vi "8-Tap 8-bit Camera with Serial Server(FPGA).vi"() -> ()   [LabVIEW 2013]
doc: "This is the FPGA VI for the 10-Tap 8-Bit Camera with DRAM example. This example demonstrates how to acquire images from a 10-tap, 8-bit, extended configuration, Camera Link camera and transfer the images to the host. This example supports area scan and line scan cameras for both continuous and finite acquisitions.\n\nThis example also demonstrates the use of DRAM as a frame buffer for very high speed acquisitions. Data packing and flow-control are also employed to maximize use of the available DRAM and FIFOs in terms of both memory space and performance.\n\nAdditionally, the example demonstrates the serial server, which allows third-party camera configuration utilities to communicate with the camera using the Camera Link serial interface while this VI is running."
uses:
  Common/CL Signal Mapping.ctl
  Common/CL Configuration.ctl
  FPGA/Sector/Accumulate/Sector Parameter Cluster.ctl
  <vilib>/Platform/TimedLoop/XDataNode/timing_clust.ctl
  <vilib>/Platform/TimedLoop/XDataNode/nitl_modes.ctl
  <vilib>/Platform/TimedLoop/XDataNode/wakeup.ctl
  <vilib>/rvi/eio/common/nirviEmuTemplateMethod_errors.vi
  <vilib>/rvi/Emulation/niFpgaSctlEmulationGetInTimedLoop.vi
  <vilib>/rvi/Emulation/niFpgaEmulationReportErrorSimple.vi
  <vilib>/rvi/Emulation/niFpgaGetClockAttributes.vi
  <vilib>/rvi/Emulation/niFpgaCriticalErrorInLSC.vi
  Common/CL Data to Pixels/8 Tap 8-Bit.vi
  FPGA/Globals/Accumulated Sector Intensity.vi
  <vilib>/rvi/FIFO/Fifo_Resource/nirvififoEmulationWriteFpgaImpl.vi
  <vilib>/rvi/DataTransferAndStorage/Container/Common/niFpgaContainerGetUniqueNameForEmu.vi
  <vilib>/rvi/interface/RandomDataEmulation/nirviRandomDataFPGAFIFO.vi
  <vilib>/rvi/interface/RandomDataEmulation/niFpgaRandomDataHandleErrors.vi
  <vilib>/rvi/FIFO/Fifo_Resource/nirvififoEmulationGetNumberOfElementsToReadFpgaImpl.vi
  <vilib>/rvi/FIFO/Fifo_Resource/nirvififoEmulationGetNumberOfElementsToWriteFpgaImpl.vi
  <vilib>/rvi/FIFO/Fifo_Resource/nirvififoEmulationReadFpgaImpl.vi
  FPGA/Globals/Sector Parameter Global.vi
  <vilib>/rvi/DataTransferAndStorage/Container/Common/niFpgaContainerExecOnDevCompGetState.vi
  <vilib>/rvi/eio/common/nirviEmuReportErrorAndStop.vi
  <vilib>/rvi/Emulation/niFpgaProcessEmulError.vi
  FPGA/Globals/Pixel Location Global.vi
  <vilib>/Platform/TimedLoop/XDataNode/XDataNode.xnode
  <vilib>/eio/EIONode/EIONode.xnode
  <vilib>/rvi/DataTransferAndStorage/Container/XNode/niFpgaContainer.xnode
  <vilib>/rvi/FIFO/Fifo_Resource/nirvififoEmulationWrite.vi
  <vilib>/rvi/interface/RandomDataEmulation/nirviRandomDataFpgaReadWriteTemplate.vi
  <vilib>/rvi/FIFO/Fifo_Resource/nirvififoEmulationGetNumberOfElementsToRead.vi
  <vilib>/rvi/FIFO/Fifo_Resource/nirvififoEmulationGetNumberOfElementsToWrite.vi
  <vilib>/rvi/FIFO/Fifo_Resource/nirvififoEmulationRead.vi
  <vilib>/rvi/FIFO/Fifo_Resource/niFpgaFifoEmulationRefIn.vi
  <vilib>/Platform/TimedLoop/XDataNode/XDNodeRunTimeDep.lvlib
panel:
  out "Host DMA Timeout":bool
  out "Logging?":bool
  in  "Consecutive Sector Threshold":u8
  out "Analysis Ticks":u32
  out "Right Sector Edge":u16
  out "Left Sector Edge":u16
  in  "# of Frames to Average":u8
  in  "Sector Parameters Left":T1={"Start Angle"=0.65740966796875, "End Angle"=0.99468994140625, "Inner Radius"=309, "Outter Radius"=405, "Hinge X"=464, "Hinge Y"=534, "NumWingSectors"=8}
  in  "Sector Parameters Right":T1={"Start Angle"=0.0, "End Angle"=0.4708251953125, "Inner Radius"=309, "Outter Radius"=405, "Hinge X"=685, "Hinge Y"=527, "NumWingSectors"=8}
  in  "Sector Threshold":u8
  in  "[Average BG Intensity]":u8[](array[numeric])=[0, 0, 0, 0, 0, 0, 0, 0, 0, 0, 0, 0, 0, 0, 0, 0, 0, 0, 0, 0, 0, 0, 0, 0, 0, 0, 0, 0, 0, 0, 0, 0]
  in  "X Resolution":u16=1000
  in  "Y Resolution":u16=1000
  in  "Left Start Angle Duty Cycle":fxp<+,8,0>
  in  "Left End Angle Duty Cycle":fxp<+,8,0>
  in  "Right Start Angle Duty Cycle":fxp<+,8,0>
  in  "Right End Angle Duty Cycle":fxp<+,8,0>
  out "Number of Elements to Write Host DMA":u32
  out "Number of Elements to Read Cam Data":u32
  in  "CL Config.Configuration":T2=enum."Full"
  in  "CL Config.Signal Mapping":T3
  in  "CL Config.Line Scan":bool
  in  "CL Config.DVAL Active High":bool=TRUE
  in  "CL Config.LVAL Active High":bool=TRUE
  in  "CL Config.FVAL Active High":bool=TRUE
  in  "CL Config.Spare Active High":bool=TRUE
  in  "Acq Control.Line Scan Height":u32
  in  "Acq Control.Frames To Acq":u32
  in  "Acq Control.Acquire":bool
  in  "Acq Control.Cancel Acq":bool
  in  "Acq Control.Ignore DVAL":bool
  in  "Acq Control.Initialize":bool
  out "Acq Status.Acq In Progress":bool
  out "Acq Status.Clocks Per Line":u32
  out "Acq Status.Frames Acq'd":u32
  out "Acq Status.Lines Per Frame":u32
  out "Acq FIFO Timeout":bool
  out "Acq Status.Initialized":bool
  in  "UART.Baud Rate":u8
  in  "UART.Transmit":bool
  in  "UART.Tx Data":u8[](array[numeric])=[0, 0, 0, 0, 0, 0, 0, 0, 0, 0] format="%02x"
  in  "UART.Set Baud Rate":bool
  in  "UART.Byte Mode":bool=TRUE
  out "UART.Rx Ready":bool
  out "UART.Break Indicator":bool
  out "UART.Framing Error":bool
  out "UART.Overrun Error":bool
  out "UART.Tx Ready":bool
  out "UART.Rx Data":u8 format="%02x"
  in  "UART.Receive":bool
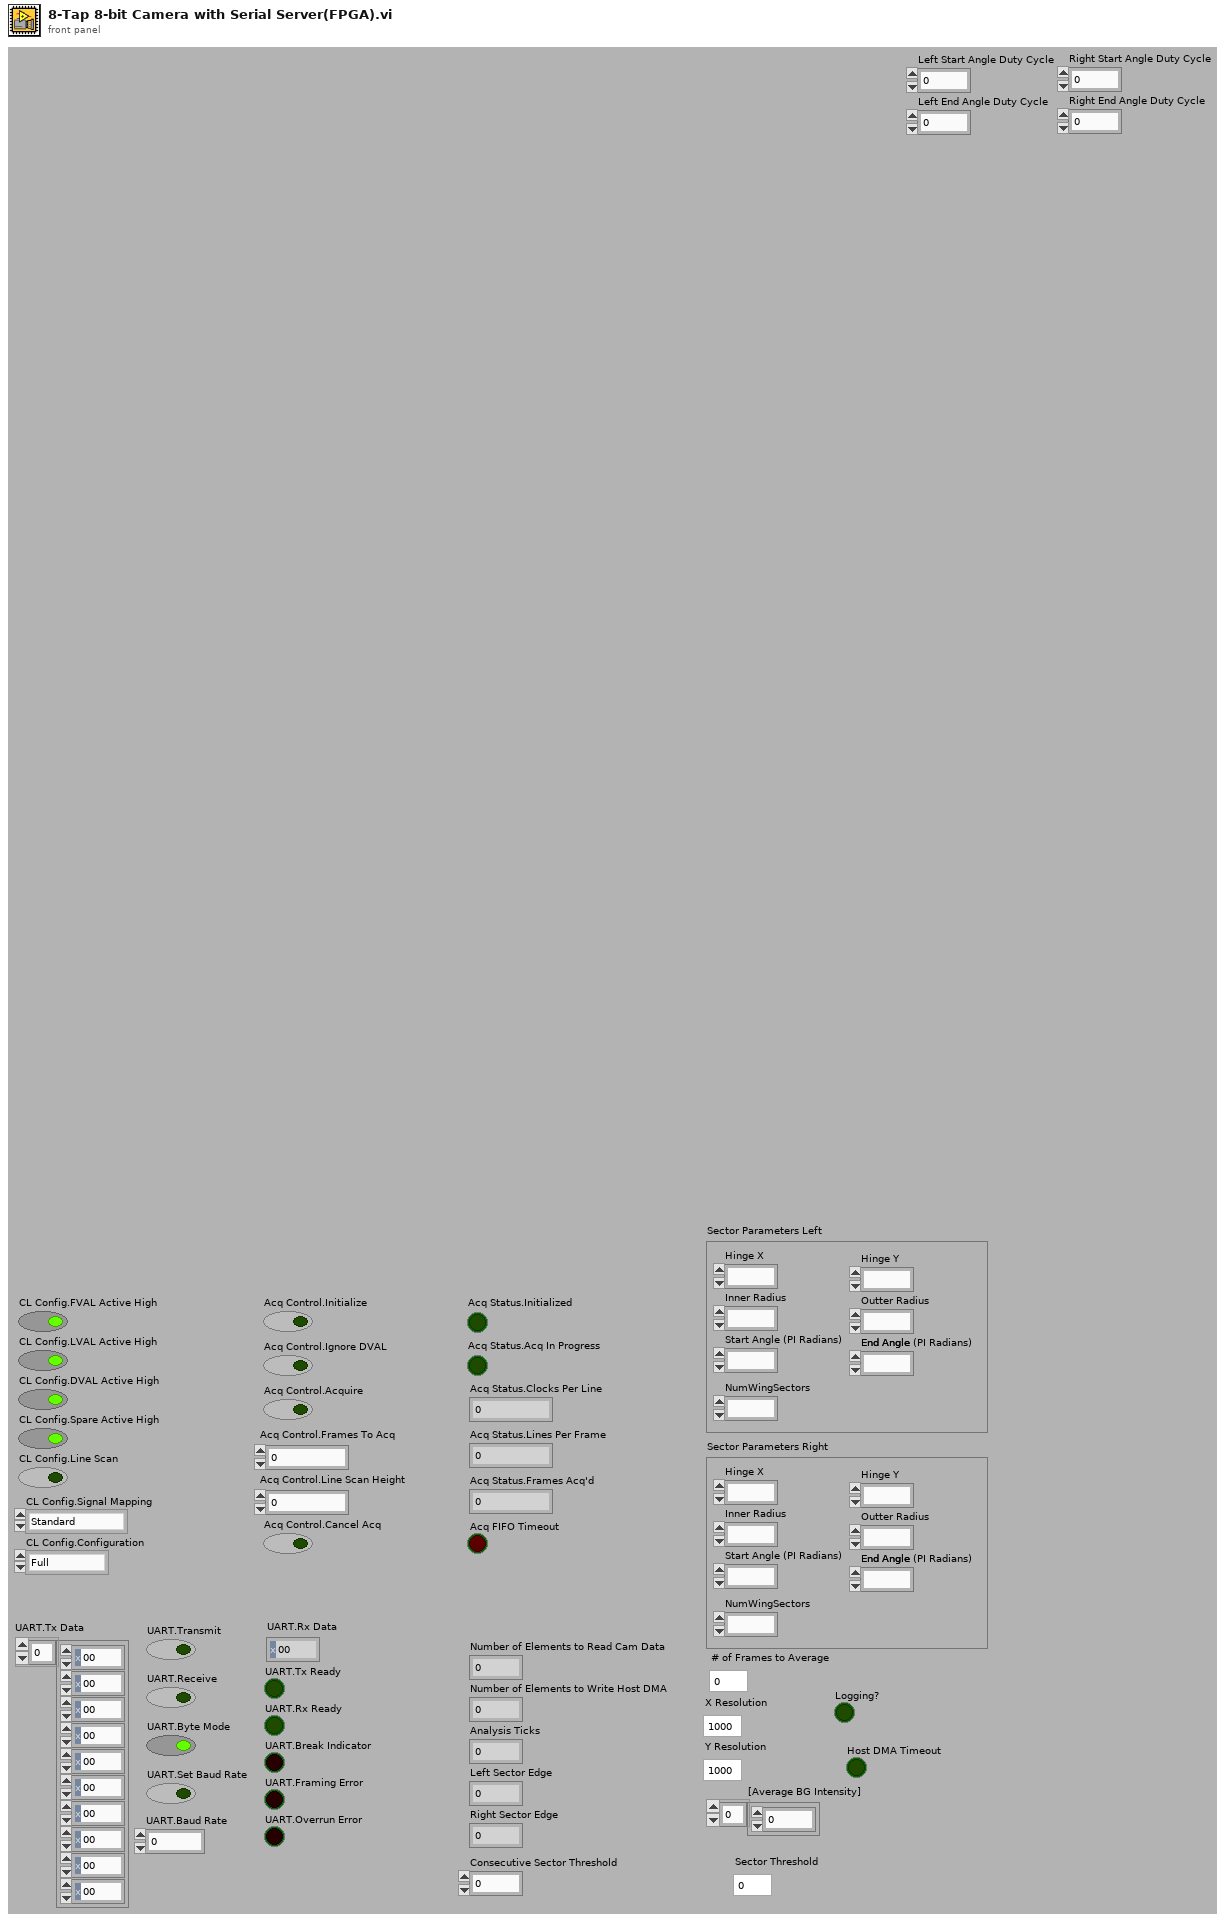
[diagram p1: front panel]
types:
  T1 = typedef "Sector Parameter Cluster.ctl" = cluster{"Start Angle":fxp<+/-,17,2>, "End Angle":fxp<+/-,17,2>, "Inner Radius":u16, "Outter Radius":u16, "Hinge X":u16, "Hinge Y":u16, "NumWingSectors":u8}
  T2 = typedef "CL Configuration.ctl" = enum8{"Base", "Medium", "Full"}
  T3 = typedef "CL Signal Mapping.ctl" = enum8{"Standard", "Basler 10-tap", "Vosskühler 10-tap"}
  T4 = typedef "XDNodeRunTimeDep.lvlib/timing_clust.ctl" = cluster{"Expected End [f-1]":u64, "Actual End [f-1]":u64, "Finished Late? [f-1]":bool, "Expected End [i-1]":u64, "Actual End [i-1]":u64, "Finished Late? [i-1]":bool, "Expected Start [i]":u64, "Actual Start [i]":u64, "Expected Start [f]":u64, "Actual Start [f]":u64, "Source Name":string, "Structure Name":string, "Period":i64, "Deadline":i64, "Offset":i64, "Start":i64, "Priority":i32, "Timeout":i32, "Mode":T5, "Wakeup Reason":T6, "Error":errorcluster, "Source Type":string, "Secondary Source Type":string, "Global End Time":u64, "Global Start Time":u64, "Frame Duration":u64, "Iteration Duration":u64, "Assigned CPU":i32, "I/O Scan Engine Mode":u32}
  T5 = typedef "XDNodeRunTimeDep.lvlib/nitl_modes.ctl" = enum32{"No Change", "Process missed periods, maintain original phase", "Discard missed periods, maintain original phase", "Process missed periods, ignore original phase", "Discard missed periods, ignore original phase"}
  T6 = typedef "XDNodeRunTimeDep.lvlib/wakeup.ctl" = enum32{"Normal", "Aborted", "Asynchronous wakeup", "Timing source error", "Timed loop error", "Timeout"}
  T7 = cluster{"Enables Valid":bool, "Frame Valid":bool, "Line Valid":bool, "Data Valid":bool}
  T8 = cluster{"Pixel 0":u8, "Pixel 1":u8, "Pixel 2":u8, "Pixel 3":u8, "Pixel 4":u8, "Pixel 5":u8, "Pixel 6":u8, "Pixel 7":u8}
  T9 = cluster{"Tx Data":u8[], "Transmit":bool, "Receive":bool, "Byte Mode":bool, "Set Baud Rate":bool, "Baud Rate":u8}
  T10 = cluster{"Rx Data":u8, "Turn Off Transmit":bool, "Turn Off Receive":bool, "Turn Off Set Baud Rate":bool, "Tx Ready":bool, "Rx Ready":bool, "Break Indicator":bool, "Framing Error":bool, "Overrun Error":bool}
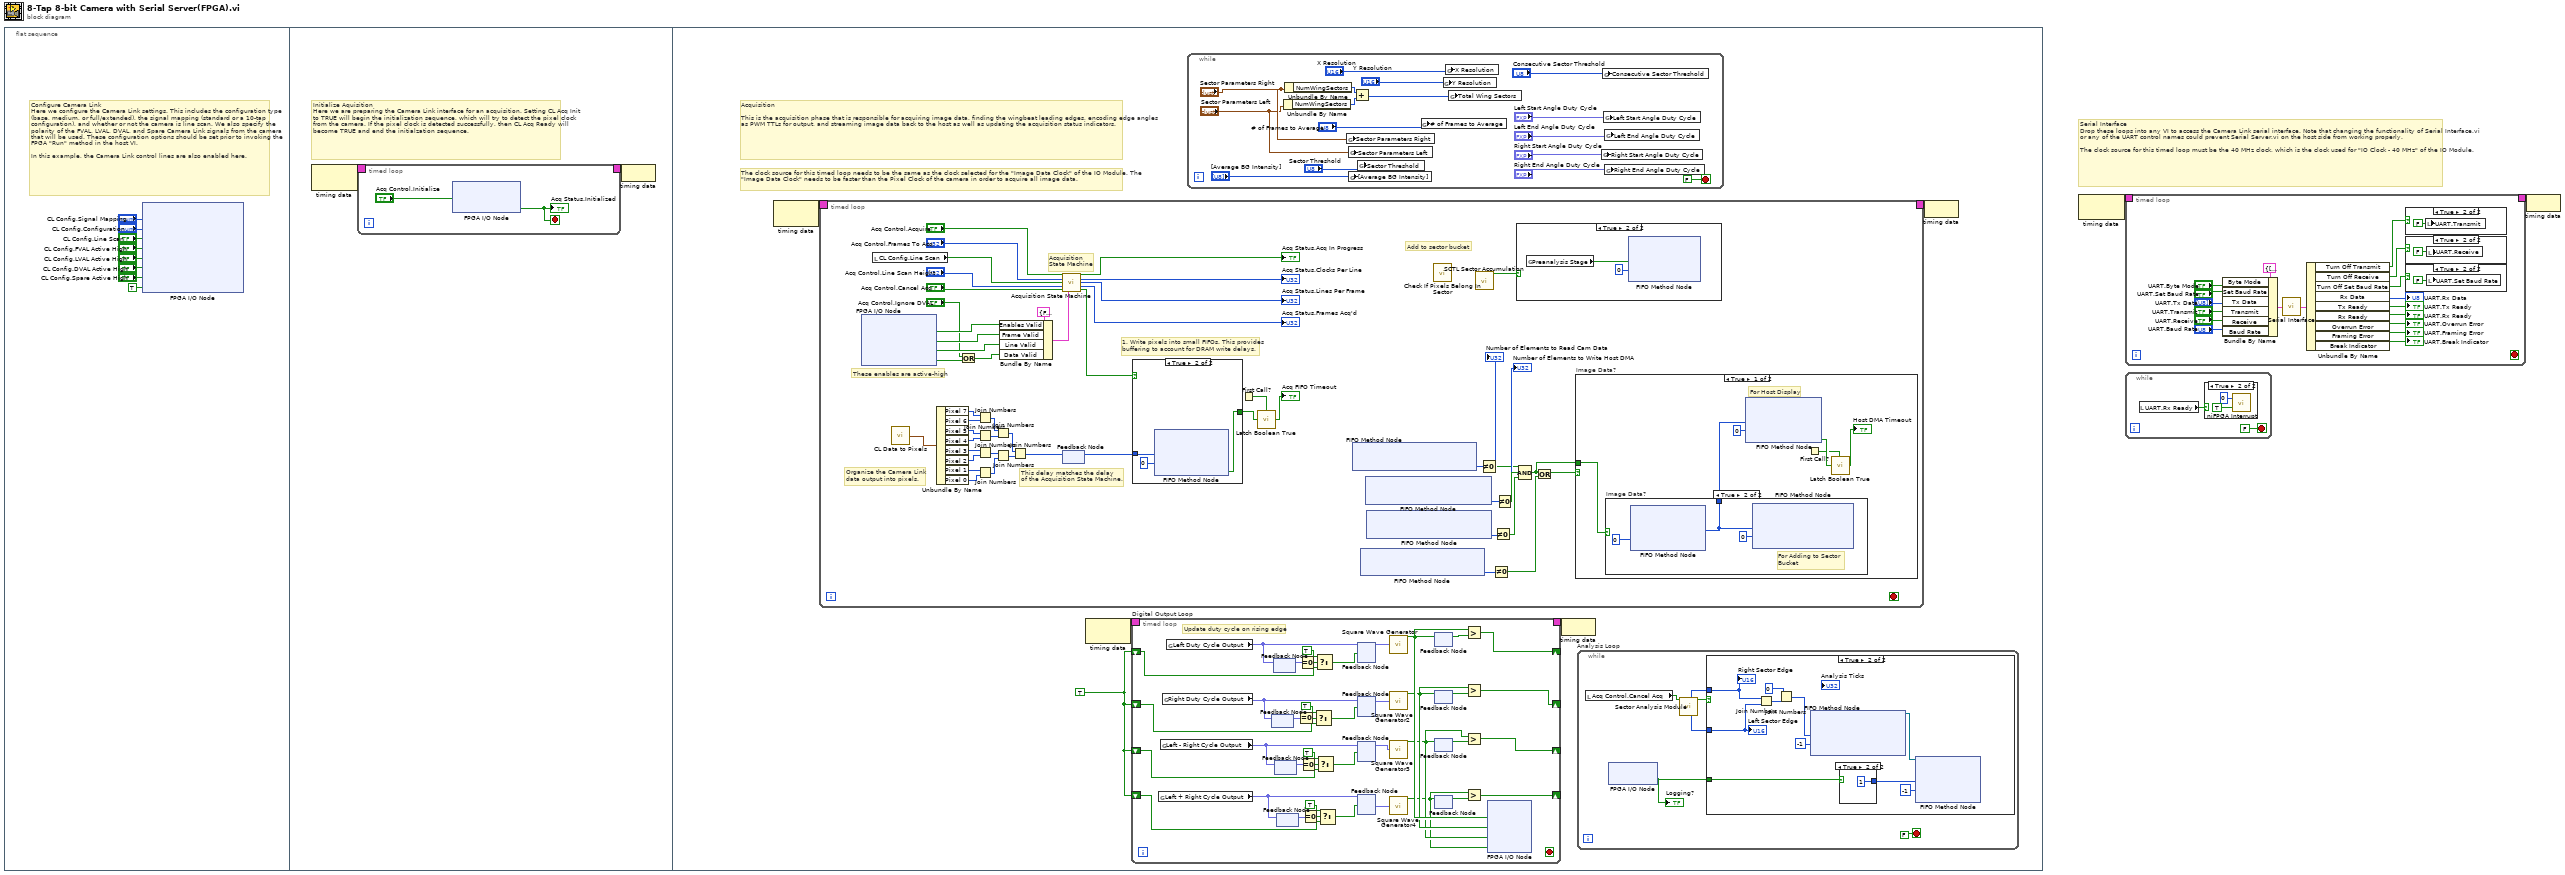
[diagram p0: block diagram]
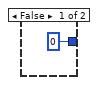
[diagram p7: hidden frame]
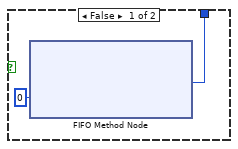
[diagram p8: hidden frame]
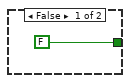
[diagram p11: hidden frame]
diagram:
  # "Serial Interface\nDrop these loops into any VI to access the Camera Link serial interface. Note that changing the functionality of Serial Interface.vi or any of the UART control names could prevent Serial Server.vi on the host side from working properly.\n\nThe clock source for this timed loop must be the 40 MHz clock, which is the clock used for \"IO Clock - 40 MHz\" of the IO Module."
  n1 = flat-sequence {
    frame #0 {
      # "Configure Camera Link\nHere we configure the Camera Link settings. This includes the configuration type (base, medium, or full/extended), the signal mapping (standard or a 10-tap configuration), and whether or not the camera is line scan. We also specify the polarity of the FVAL, LVAL, DVAL, and Spare Camera Link signals from the camera that will be used. These configuration options should be set prior to invoking the FPGA \"Run\" method in the host VI.\n\nIn this example, the Camera Link control lines are also enabled here."
      n2 = xnode "FPGA I/O Node"("CL Set Signal Mapping"="CL Config.Signal Mapping", "CL Set Configuration"="CL Config.Configuration", "CL Set Line Scan"="CL Config.Line Scan", "CL Set FVAL Active High"="CL Config.FVAL Active High", "CL Set LVAL Active High"="CL Config.LVAL Active High", "CL Set DVAL Active High"="CL Config.DVAL Active High", "CL Set Spare Active High"="CL Config.Spare Active High", "CL Control Enable"=TRUE ("IO Module\\CL Control Enable")) -> ()  [unwired: 8 in, 8 out]
    }
    frame #1 {
      # "Initialize Aquisition\nHere we are preparing the Camera Link interface for an acquisition. Setting CL Acq Init to TRUE will begin the initialization sequence, which will try to detect the pixel clock from the camera. If the pixel clock is detected successfully, then CL Acq Ready will become TRUE and end the initialzation sequence."
      n3 = node-c288() -> (w12:T4)  [unwired: 1 out]
      n4 = timed-loop {
        timing: w12 -> [_]
        timing-out: [_] -> w11
        stop <- w13 stop-if-true
        n5 = xnode "FPGA I/O Node"("CL Acq Init"="Acq Control.Initialize") -> ("CL Acq Ready"=w13:bool)  [unwired: 2 in, 2 out]
        "Acq Status.Initialized" <- w13
      }
      n6 = node-c288(w11) -> ()
    }
    frame #2 {
      w19 = TRUE
      # "The clock source for this timed loop needs to be the same as the clock selected for the \"Image Data Clock\" of the IO Module. The \"Image Data Clock\" needs to be faster than the Pixel Clock of the camera in order to acquire all image data."
      # "Acquisition\n\nThis is the acquisition phase that is responsible for acquiring image data, finding the wingbeat leading edges, encoding edge angles as PWM TTLs for output, and streaming image data back to the host as well as updating the acquisition status indicators."
      n7 = node-c288() -> (w23:T4)  [unwired: 1 in]
      n8 = timed-loop {
        timing: w23 -> [_]
        timing-out: [_] -> w22
        stop <- _ stop-if-true
        # "Add to sector bucket"
        # "1. Write pixels into small FIFOs. This provides\nbuffering to account for DRAM write delays."
        # "Organize the Camera Link\ndata output into pixels."
        # "These enables are active-high"
        # "This delay matches the delay\nof the Acquisition State Machine."
        # "Acquisition\nState Machine"
        n9 = xnode "FPGA I/O Node"() -> ("CL Output Valid"=w140:bool, "CL Frame Valid"=w139:bool, "CL Line Valid"=w138:bool, "CL Data Valid"=w135:bool)  [unwired: 4 in, 4 out]
        n10 = local read "CL Config.Line Scan"() -> (w132:bool)
        n11 = call-poly "CL Data to Pixels.vi"() -> ("Pixels"=w150:T8)  [unwired: 1 in]
        n12 = Unbundle By Name(w150) -> ("Pixel 7"=w130:u8, "Pixel 6"=w129:u8, "Pixel 5"=w128:u8, "Pixel 4"=w127:u8, "Pixel 3"=w126:u8, "Pixel 2"=w125:u8, "Pixel 1"=w124:u8, "Pixel 0"=w123:u8)
        n13 = Or(x="Acq Control.Ignore DVAL", y=w135) -> (x .or. y?=w134:bool)
        n14 = Join Numbers(hi=w130, lo=w129) -> ((hi.lo)=w121:u16)
        n15 = Join Numbers(hi=w128, lo=w127) -> ((hi.lo)=w120:u16)
        n16 = Join Numbers(hi=w126, lo=w125) -> ((hi.lo)=w119:u16)
        n17 = Join Numbers(hi=w124, lo=w123) -> ((hi.lo)=w122:u16)
        n18 = Join Numbers(hi=w121, lo=w120) -> ((hi.lo)=w118:u32)
        n19 = Join Numbers(hi=w119, lo=w122) -> ((hi.lo)=w117:u32)
        n20 = Bundle By Name(cluster=T7 {"Enables Valid"=FALSE, "Frame Valid"=FALSE, "Line Valid"=FALSE, "Data Valid"=FALSE} ("Enables"), "Enables Valid"=w140, "Frame Valid"=w139, "Line Valid"=w138, "Data Valid"=w134) -> (w137:T7)
        n21 = Join Numbers(hi=w118, lo=w117) -> ((hi.lo)=w116:u64)
        n22 = call "Acquisition State Machine.vi"("Acquire"="Acq Control.Acquire", "Frames to Acquire"="Acq Control.Frames To Acq", "Line Scan"=w132, "Line Scan Height"="Acq Control.Line Scan Height", "Cancel Acq"="Acq Control.Cancel Acq", "Enables"=w137) -> ("Acq In Progress"=→"Acq Status.Acq In Progress":bool, "Num Clocks Per Line"=→"Acq Status.Clocks Per Line":u32, "Num Lines Per Frame"=→"Acq Status.Lines Per Frame":u32, "Num Frames Acq'd"=→"Acq Status.Frames Acq'd":u32, "Capture Cycle"=w148:bool)  [unwired: 4 in, 1 out]
        n23 = feedback-in #1(w116) -> ()
        n24 = feedback #1() -> (w149:u64)  [unwired: 1 in]
        n25 = case shown="True" w148 {
          tunnel: [FALSE ("Timed Out?") w166] -> w104
          tunnel: w149 -> [_ w167]
          frame False {
          }
          frame True {
            n26 = xnode ("FIFO Method Node")("Element"=w167, "Timeout"=0) -> ("Timed Out?"=w166:bool)  [unwired: 1 in, 1 out]
          }
        }
        n27 = First Call?() -> (First Call?: T/F=w103:bool)
        n28 = call "Latch Boolean True.vi"("Input"=w104, "Reset?"=w103) -> ("Latched True"=→"Acq FIFO Timeout":bool)
        n29 = xnode ("FIFO Method Node")() -> ("Number of Elements to Read"=w114:u32)  [unwired: 1 in, 1 out]
        "Number of Elements to Read Cam Data" <- w114
        n30 = xnode ("FIFO Method Node")() -> ("Number of Elements to Read"=w108:u32)  [unwired: 1 in, 1 out]
        n31 = xnode ("FIFO Method Node")() -> ("Number of Elements to Write"=w112:u32)  [unwired: 1 in, 1 out]
        "Number of Elements to Write Host DMA" <- w112
        n32 = xnode ("FIFO Method Node")() -> ("Number of Elements to Write"=w111:u32)  [unwired: 1 in, 1 out]
        n33 = call "Check If Pixels Belong In Sector.vi"() -> ()  [unwired: 11 in, 1 out]
        n34 = call "SCTL Sector Accumulation.vi"() -> ("New Data?"=w115:bool)  [unwired: 10 in, 1 out]
        n35 = Not Equal To 0?(x=w114) -> (x != 0?=w109:bool)
        n36 = Not Equal To 0?(x=w108) -> (x != 0?=w106:bool)
        n37 = Not Equal To 0?(x=w111) -> (x != 0?=w110:bool)
        n38 = Not Equal To 0?(x=w112) -> (x != 0?=w113:bool)
        n39 = case shown="True" w115 {
          frame False {
          }
          frame True {
            n40 = global read "Accumulated Sector Intensity.vi" "Preanalysis Stage"() -> (w162:bool)
            n41 = xnode ("FIFO Method Node")("Element"=w162, "Timeout"=0) -> ()  [unwired: 1 in, 2 out]
          }
        }
        n42 = Compound Arithmetic op=AND(w109, w113, w110) -> (w105:bool)
        n43 = Or(x=w105, y=w106) -> (x .or. y?=w107:bool)
        n44 = case "Image Data?" shown="True" w107 {
          tunnel: w105 -> [w154 _]
          frame True {
            # "For Host Display"
            n45 = case "Image Data?" shown="True" w154 {
              tunnel: [w158 w161] -> w155
              frame False {
                n46 = xnode ("FIFO Method Node")("Timeout"=0) -> ("Element"=w158:u64)  [unwired: 1 in, 2 out]
              }
              frame True {
                # "For Adding to Sector \nBucket"
                n47 = xnode ("FIFO Method Node")("Timeout"=0) -> ("Element"=w161:u64)  [unwired: 1 in, 2 out]
                n48 = xnode ("FIFO Method Node")("Element"=w161, "Timeout"=0) -> ()  [unwired: 1 in, 2 out]
              }
            }
            n49 = xnode ("FIFO Method Node")("Element"=w155, "Timeout"=0) -> ("Timed Out?"=w153:bool)  [unwired: 1 in, 1 out]
            n50 = First Call?() -> (First Call?: T/F=w152:bool)
            n51 = call "Latch Boolean True.vi"("Input"=w153, "Reset?"=w152) -> ("Latched True"=→"Host DMA Timeout":bool)
          }
          frame False {
          }
        }
      }
      n52 = node-c288() -> (w21:T4)  [unwired: 1 in]
      n53 = timed-loop "Digital Output Loop" {
        timing: w21 -> [_]
        timing-out: [_] -> w20
        shift-right: [w91] -> _
        shift-left: w19 -> [w76]
        shift-right: [w90] -> _
        shift-left: w19 -> [w62]
        shift-right: [w89] -> _
        shift-left: w19 -> [w60]
        shift-right: [w83] -> _
        shift-left: w19 -> [w58]
        stop <- _ stop-if-true
        # "Update duty cycle on rising edge"
        n54 = global read "Sector Parameter Global.vi" "Left + Right Cycle Output"() -> (w64:fxp<+,8,0>)
        n55 = global read "Sector Parameter Global.vi" "Left - Right Cycle Output"() -> (w65:fxp<+,8,0>)
        n56 = global read "Sector Parameter Global.vi" "Right Duty Cycle Output"() -> (w66:fxp<+/-,9,1>)
        n57 = global read "Sector Parameter Global.vi" "Left Duty Cycle Output"() -> (w79:fxp<+/-,9,1>)
        n58 = feedback #2() -> (w73:fxp<+/-,9,1>)  [unwired: 1 in]
        n59 = feedback-in #2(w66) -> ()
        n60 = feedback #3() -> (w78:fxp<+/-,9,1>)  [unwired: 1 in]
        n61 = feedback-in #3(w79) -> ()
        n62 = feedback #4() -> (w70:fxp<+,8,0>)  [unwired: 1 in]
        n63 = feedback-in #4(w65) -> ()
        n64 = feedback #5() -> (w67:fxp<+,8,0>)  [unwired: 1 in]
        n65 = feedback-in #5(w64) -> ()
        n66 = Equal To 0?(x=w73) -> (x = 0?=w74:bool)
        n67 = Equal To 0?(x=w78) -> (x = 0?=w80:bool)
        n68 = Equal To 0?(x=w70) -> (x = 0?=w71:bool)
        n69 = Equal To 0?(x=w67) -> (x = 0?=w68:bool)
        n70 = Select(t=TRUE, s=w74, f=w62) -> (s? t:f=w63:bool)
        n71 = Select(t=TRUE, s=w80, f=w76) -> (s? t:f=w77:bool)
        n72 = Select(t=TRUE, s=w71, f=w60) -> (s? t:f=w61:bool)
        n73 = Select(t=TRUE, s=w68, f=w58) -> (s? t:f=w59:bool)
        n74 = feedback-in #6(w79, w77) -> ()
        n75 = feedback #6() -> (w97:fxp<+/-,9,1>)  [unwired: 1 in]
        n76 = feedback #7() -> (w96:fxp<+/-,9,1>)  [unwired: 1 in]
        n77 = feedback-in #7(w66, w63) -> ()
        n78 = feedback #8() -> (w95:fxp<+,8,0>)  [unwired: 1 in]
        n79 = feedback-in #8(w65, w61) -> ()
        n80 = feedback #9() -> (w85:fxp<+,8,0>)  [unwired: 1 in]
        n81 = feedback-in #9(w64, w59) -> ()
        n82 = call "Square Wave Generator"("duty cycle (periods)"=w97) -> ("square wave out"=w88:bool)  [unwired: 14 in]
        n83 = call "Square Wave Generator2"("duty cycle (periods)"=w96) -> ("square wave out"=w87:bool)  [unwired: 14 in]
        n84 = call "Square Wave Generator3"("duty cycle (periods)"=w95) -> ("square wave out"=w86:bool)  [unwired: 14 in]
        n85 = call "Square Wave Generator4"("duty cycle (periods)"=w85) -> ("square wave out"=w82:bool)  [unwired: 14 in]
        n86 = feedback-in #10(w88) -> ()
        n87 = feedback #10() -> (w94:bool)  [unwired: 1 in]
        n88 = feedback #11() -> (w93:bool)  [unwired: 1 in]
        n89 = feedback-in #11(w87) -> ()
        n90 = feedback #12() -> (w92:bool)  [unwired: 1 in]
        n91 = feedback-in #12(w86) -> ()
        n92 = feedback #13() -> (w84:bool)  [unwired: 1 in]
        n93 = feedback-in #13(w82) -> ()
        n94 = Greater?(x=w88, y=w94) -> (0:w91:bool)
        n95 = Greater?(x=w87, y=w93) -> (0:w90:bool)
        n96 = Greater?(x=w86, y=w92) -> (0:w89:bool)
        n97 = Greater?(x=w82, y=w84) -> (0:w83:bool)
        n98 = xnode "FPGA I/O Node"("TTL 1"=w88, "TTL 2"=w87, "TTL 3"=w86, "TTL 4"=w82) -> ()  [unwired: 4 in, 4 out]
      }
      n99 = while {
        stop <- FALSE stop-if-true
        n100 = Unbundle By Name("Sector Parameters Left") -> ("NumWingSectors"=w55:u8)
        n101 = Unbundle By Name("Sector Parameters Right") -> ("NumWingSectors"=w56:u8)
        n102 = global write "Sector Parameter Global.vi" "Sector Parameters Right"("Sector Parameters Right") -> ()
        n103 = global write "Sector Parameter Global.vi" "Sector Parameters Left"("Sector Parameters Left") -> ()
        n104 = global write "Sector Parameter Global.vi" "[Average BG Intensity]"("[Average BG Intensity]") -> ()
        n105 = Add(x=w56, y=w55) -> (x+y=w54:u8)
        n106 = global write "Sector Parameter Global.vi" "Sector Threshold"("Sector Threshold") -> ()
        n107 = global write "Pixel Location Global.vi" "# of Frames to Average"("# of Frames to Average") -> ()
        n108 = global write "Pixel Location Global.vi" "Y Resolution"("Y Resolution") -> ()
        n109 = global write "Pixel Location Global.vi" "X Resolution"("X Resolution") -> ()
        n110 = global write "Accumulated Sector Intensity.vi" "Total Wing Sectors"(w54) -> ()
        n111 = global write "Sector Parameter Global.vi" "Right Start Angle Duty Cycle"("Right Start Angle Duty Cycle") -> ()
        n112 = global write "Sector Parameter Global.vi" "Consecutive Sector Threshold"("Consecutive Sector Threshold") -> ()
        n113 = global write "Sector Parameter Global.vi" "Left Start Angle Duty Cycle"("Left Start Angle Duty Cycle") -> ()
        n114 = global write "Sector Parameter Global.vi" "Left End Angle Duty Cycle"("Left End Angle Duty Cycle") -> ()
        n115 = global write "Sector Parameter Global.vi" "Right End Angle Duty Cycle"("Right End Angle Duty Cycle") -> ()
      }
      n116 = node-c288(w20) -> ()
      n117 = while "Analysis Loop" {
        stop <- FALSE stop-if-true
        n118 = local read "Acq Control.Cancel Acq"() -> (w28:bool)
        n119 = xnode "FPGA I/O Node"() -> ("ISO In 0"=w24:bool)  [unwired: 1 in, 1 out]
        "Logging?" <- w24
        n120 = call "Sector Analysis Module.vi"("Canceled?"=w28) -> ("Data"=w25:bool, "Left Sector Edge"=w26:u16, "Right Sector Edge"=w27:u16)  [unwired: 7 in, 1 out]
        n121 = case shown="True" w25 {
          tunnel: w27 -> [_ w39]
          tunnel: w26 -> [_ w38]
          tunnel: w24 -> [_ w32]
          frame False {
          }
          frame True {
            n122 = Join Numbers(hi=w39, lo=w38) -> ((hi.lo)=w37:u32)
            n123 = Join Numbers(hi=u32 0, lo=w37) -> ((hi.lo)=w35:u64)
            n124 = xnode ("FIFO Method Node")("Element"=w35, "Timeout"=-1) -> ("FIFO Out"=w33:refnum<k21>)  [unwired: 1 in, 1 out]
            n125 = case shown="True" w32 {
              tunnel: [u64 0 ("Element") u64 1 ("Element")] -> w31
              frame False {
              }
              frame True {
              }
            }
            n126 = xnode ("FIFO Method Node")("Element"=w31, "Timeout"=-1, "FIFO In"=w33) -> ()  [unwired: 2 out]
            "Right Sector Edge" <- w39
            "Left Sector Edge" <- w38
          }
        }
      }
      n127 = node-c288(w22) -> ()
    }
  }
  n128 = node-c288() -> (w2:T4)  [unwired: 1 out]
  n129 = timed-loop {
    timing: w2 -> [_]
    timing-out: [_] -> w1
    stop <- _ stop-if-true
    n130 = Bundle By Name(cluster=T9 {"Tx Data"=[0, 0, 0, 0, 0, 0, 0, 0, 0, 0], "Transmit"=FALSE, "Receive"=FALSE, "Byte Mode"=TRUE, "Set Baud Rate"=FALSE, "Baud Rate"=0} ("UART Inputs"), "Byte Mode"="UART.Byte Mode", "Set Baud Rate"="UART.Set Baud Rate", "Tx Data"="UART.Tx Data", "Transmit"="UART.Transmit", "Receive"="UART.Receive", "Baud Rate"="UART.Baud Rate") -> (w172:T9)
    n131 = call "Serial Interface.vi"("UART Inputs"=w172) -> ("UART Outputs"=w184:T10)
    n132 = Unbundle By Name(w184) -> ("Turn Off Transmit"=w177:bool, "Turn Off Receive"=w178:bool, "Turn Off Set Baud Rate"=w174:bool, "Rx Data"=→"UART.Rx Data":u8, "Tx Ready"=→"UART.Tx Ready":bool, "Rx Ready"=→"UART.Rx Ready":bool, "Overrun Error"=→"UART.Overrun Error":bool, "Framing Error"=→"UART.Framing Error":bool, "Break Indicator"=→"UART.Break Indicator":bool)
    n133 = case shown="True" w177 {
      frame False {
      }
      frame True {
        n134 = local write "UART.Transmit"(FALSE ("UART.Transmit")) -> ()
      }
    }
    n135 = case shown="True" w178 {
      frame False {
      }
      frame True {
        n136 = local write "UART.Receive"(FALSE ("UART.Receive")) -> ()
      }
    }
    n137 = case shown="True" w174 {
      frame False {
      }
      frame True {
        n138 = local write "UART.Set Baud Rate"(FALSE ("UART.Receive")) -> ()
      }
    }
  }
  n139 = while {
    stop <- FALSE stop-if-true
    n140 = local read "UART.Rx Ready"() -> (w196:bool)
    n141 = case shown="True" w196 {
      frame False {
      }
      frame True {
        n142 = call <vilib>:"niFPGA Interrupt.vi"("Wait Until Cleared (F)"=TRUE ("Wait Until Cleared"), "IRQ Number (0)"=u8 0 ("IRQ Number")) -> ()  [unwired: 1 in]
      }
    }
  }
  n143 = node-c288(w1) -> ()
